vi "Control Inputs (SubVI).vi"(6 "Enable Kinect Extention":bool, 7 "Keyboard ID":refnum<k1>, 8 "error in (no error)":errorcluster, 9 "Switch control":bool, 10 "Manual":bool=TRUE, 11 "Controller ID":refnum<k1>) -> (0 "error out":errorcluster, 1 "Land/Take off":bool, 2 "Hover Out":bool, 3 "Control cluster":T1)   [LabVIEW 2014]
uses:
  Global.vi
panel:
  out "x-y":u32
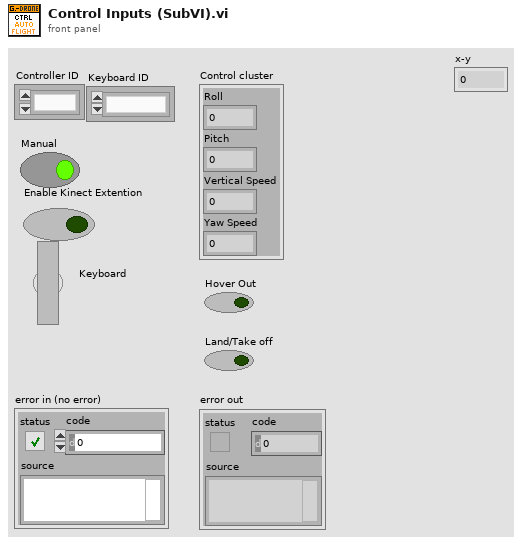
[diagram p1: front panel]
types:
  T1 = cluster{"Roll":dbl, "Pitch":dbl, "Vertical Speed":dbl, "Yaw Speed":dbl}
  T2 = cluster{"Hover":bool, "Land/Take off":bool, "button 3":bool, "button 4":bool}
  T3 = typedef "Control cluster.ctl" = cluster{"Roll":sgl, "Pitch":sgl, "Vertical Speed":sgl, "Yaw Speed":sgl}
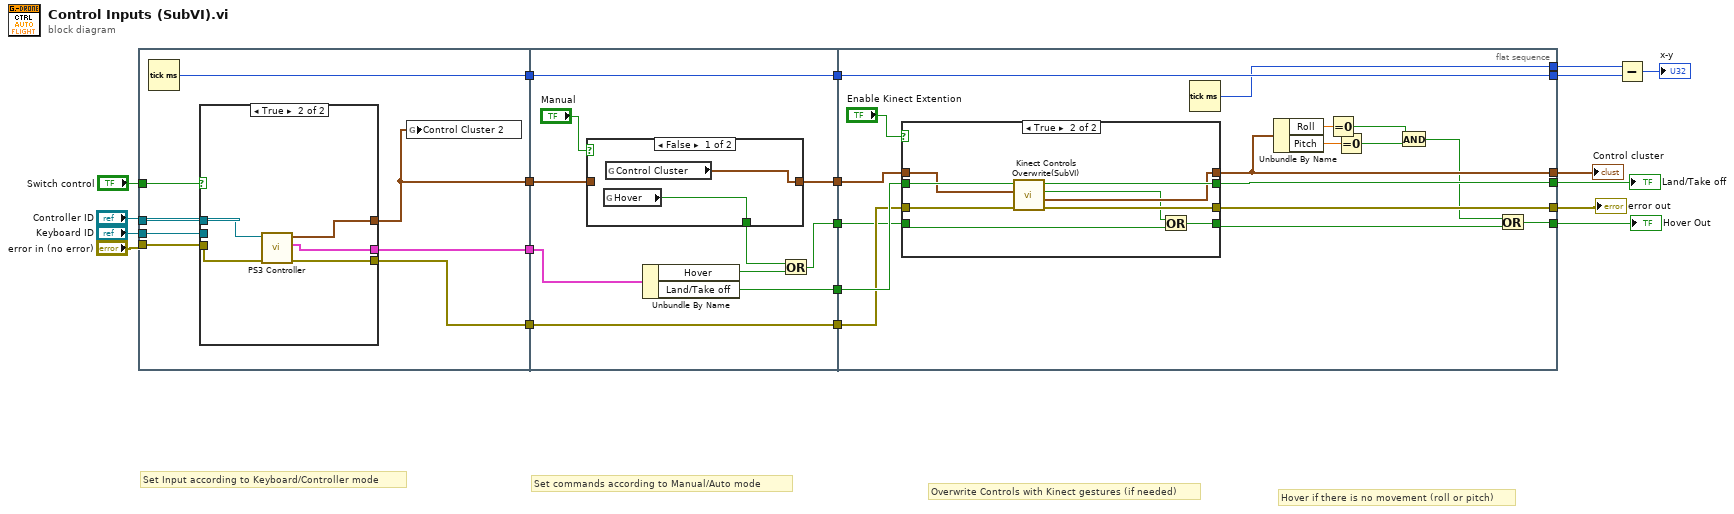
[diagram p0: block diagram]
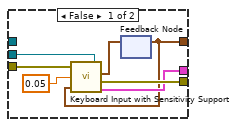
[diagram p2: hidden frame]
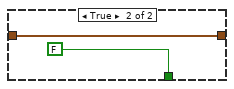
[diagram p3: hidden frame]
diagram:
  # "Hover if there is no movement (roll or pitch)"
  # "Overwrite Controls with Kinect gestures (if needed)"
  # "Set Input according to Keyboard/Controller mode"
  # "Set commands according to Manual/Auto mode"
  n1 = flat-sequence {
    tunnel: [w26] -> w16
    tunnel: [w27] -> w15
    tunnel: "error in (no error)" -> [w28]
    tunnel: "Keyboard ID" -> [w25]
    tunnel: "Controller ID" -> [w24]
    tunnel: "Switch control" -> [w23]
    tunnel: [w22] -> w9
    tunnel: [w21] -> w1
    tunnel: [w49] -> w20
    tunnel: [w47] -> w19
    tunnel: [w43] -> w18
    tunnel: [w42] -> w17
    tunnel: w16 -> [w46]
    tunnel: w15 -> [w43]
    tunnel: [w41] -> w10
    tunnel: w9 -> [w41]
    tunnel: w1 -> [w50]
    tunnel: w20 -> [w71]
    tunnel: w19 -> [w65]
    tunnel: w18 -> [w69]
    tunnel: [w68] -> w3
    tunnel: [w58] -> w5
    tunnel: w17 -> [w67]
    tunnel: [w57] -> w2
    tunnel: [w66] -> w4
    tunnel: [w64] -> w6
    tunnel: w10 -> [w64]
    tunnel: [w63] -> w7
    frame #0 {
      n2 = Tick Count (ms)() -> (millisecond timer value=w22:u32)
      n3 = case shown="True" w23 {
        tunnel: w28 -> [w35 w40]
        tunnel: [w34 w39] -> w27
        tunnel: [w30 w38] -> w21
        tunnel: [w33 w36] -> w26
        tunnel: w25 -> [w32 _]
        tunnel: w24 -> [_ w37]
        frame False {
          n4 = feedback #1() -> (w30:T1)  [unwired: 1 in]
          n5 = call "Keyboard Input with Sensitivity Support.vi"("error in (no error)"=w35, "Speed step"=0.05, "Previous Control Cluster"=w30, "device ID"=w32) -> ("Control Cluster"=w31:T1, "error out"=w34:errorcluster, "Buttons control"=w33:T2)
          n6 = feedback-in #1(w31) -> ()
        }
        frame True {
          n7 = call "PS3 Controller.vi"("error in (no error)"=w40, "device ID"=w37) -> ("error out"=w39:errorcluster, "Buttons control"=w36:T2, "Control cluster"=w38:T1)  [unwired: 7 in]
        }
      }
      n8 = global write "Global.vi" "Control Cluster 2"(w21) -> ()
    }
    frame #1 {
      n9 = case shown="False" "Manual" {
        tunnel: w50 -> [_ w53]
        tunnel: [w52 w53] -> w47
        tunnel: [w51 FALSE] -> w44
        frame False {
          n10 = global read "Global.vi" "Hover"() -> (w51:bool)
          n11 = global read "Global.vi" "Control Cluster"() -> (w52:T3)
        }
        frame True {
        }
      }
      n12 = Unbundle By Name(w46) -> ("Hover"=w45:bool, "Land/Take off"=w49:bool)
      n13 = Or(x=w44, y=w45) -> (x .or. y?=w42:bool)
    }
    frame #2 {
      n14 = case shown="True" "Enable Kinect Extention" {
        tunnel: w71 -> [w75 w84]
        tunnel: [w75 w83] -> w66
        tunnel: [w74 w82] -> w68
        tunnel: w69 -> [w74 w81]
        tunnel: w67 -> [w73 w76]
        tunnel: [w73 w78] -> w56
        tunnel: w65 -> [w72 w80]
        tunnel: [w72 w79] -> w58
        frame False {
        }
        frame True {
          n15 = call "Kinect Controls Overwrite(SubVI).vi"("error in (no error)"=w81, "Control cluster In"=w80, "Land/Take off In"=w84) -> ("error out"=w82:errorcluster, "Control cluster Out"=w79:T1, "Hover Out"=w77:bool, "Land/take off Out"=w83:bool)  [unwired: 5 in]
          n16 = Or(x=w77, y=w76) -> (x .or. y?=w78:bool)
        }
      }
      n17 = Tick Count (ms)() -> (millisecond timer value=w63:u32)
      n18 = Unbundle By Name(w58) -> ("Roll"=w62:dbl, "Pitch"=w61:dbl)
      n19 = Equal To 0?(x=w62) -> (x = 0?=w59:bool)
      n20 = Equal To 0?(x=w61) -> (x = 0?=w60:bool)
      n21 = And(x=w59, y=w60) -> (x .and. y?=w55:bool)
      n22 = Or(x=w55, y=w56) -> (x .or. y?=w57:bool)
    }
  }
  n23 = Subtract(x=w7, y=w6) -> (x-y=→"x-y":u32)
  "error out" <- w3
  "Control cluster" <- w5
  "Land/Take off" <- w4
  "Hover Out" <- w2
